vi "Estimate Charge.vi"(0 "OCV (V)":dbl, 5 "Chemistry":T1(ring)=enum."Alkaline", 11 "error in":errorcluster) -> (4 "Charge (%)":dbl, 15 "error out":errorcluster)   [LabVIEW 2026]
doc: "Approximate state of charge of an AA cell from its resting open-circuit voltage. Alkaline and Ni-MH: linear interpolation of the chemistry's OCV table (spec 'Charge estimate'), clamped to 0..100 %; an OCV below the first table point gives 0 %, above the last 100 %. Depleted gives 0 %. Every other chemistry (No Battery, Reversed Polarity, Alkaline or Ni-MH, Li-ion 1.5V (BMS), Unknown) gives NaN. Pure function: error in is passed to error out unchanged."
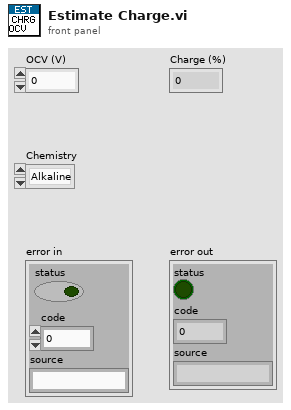
[diagram p1: front panel]
types:
  T1 = enum16{"No Battery", "Reversed Polarity", "Alkaline", "Ni-MH", "Alkaline or Ni-MH", "Li-ion 1.5V (BMS)", "Depleted", "Unknown"}
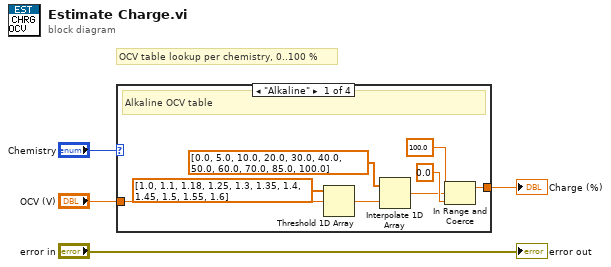
[diagram p0: block diagram]
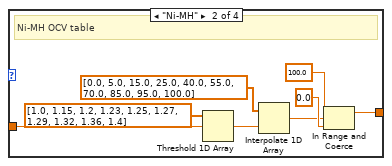
[diagram p2: hidden frame]
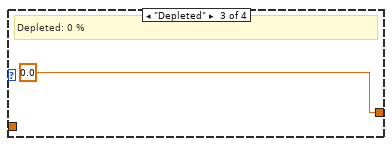
[diagram p3: hidden frame]
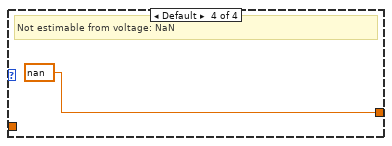
[diagram p4: hidden frame]
diagram:
  # "OCV table lookup per chemistry, 0..100 %"
  n1 = case shown="\"Alkaline\"" "Chemistry" {
    tunnel: "OCV (V)" -> [w5 w13 _ _]
    tunnel: [w12 w20 0.0 ("empty") nan ("not available")] -> w4
    frame "Alkaline" {
      # "Alkaline OCV table"
      n2 = Threshold 1D Array(2:w5, 3:dbl[] [1.0, 1.1, 1.18, 1.25, 1.3, 1.35, 1.4, 1.45, 1.5, 1.55, 1.6] ("Alkaline OCV (V)")) -> (0:w8:dbl)  [unwired: 1 in]
      n3 = Interpolate 1D Array(1:w8, 2:dbl[] [0.0, 5.0, 10.0, 20.0, 30.0, 40.0, 50.0, 60.0, 70.0, 85.0, 100.0] ("Alkaline charge (%)")) -> (0:w9:dbl)
      n4 = In Range and Coerce(upper limit=100.0, x=w9, lower limit=0.0) -> (coerced(x)=w12:dbl)  [unwired: 1 out]
    }
    frame "Ni-MH" {
      # "Ni-MH OCV table"
      n5 = Threshold 1D Array(2:w13, 3:dbl[] [1.0, 1.15, 1.2, 1.23, 1.25, 1.27, 1.29, 1.32, 1.36, 1.4] ("Ni-MH OCV (V)")) -> (0:w16:dbl)  [unwired: 1 in]
      n6 = Interpolate 1D Array(1:w16, 2:dbl[] [0.0, 5.0, 15.0, 25.0, 40.0, 55.0, 70.0, 85.0, 95.0, 100.0] ("Ni-MH charge (%)")) -> (0:w17:dbl)
      n7 = In Range and Coerce(upper limit=100.0, x=w17, lower limit=0.0) -> (coerced(x)=w20:dbl)  [unwired: 1 out]
    }
    frame "Depleted" {
      # "Depleted: 0 %"
    }
    frame Default {
      # "Not estimable from voltage: NaN"
    }
  }
  "Charge (%)" <- w4
  "error out" <- "error in"
